vi "Update Methods Registration.vi"(8 "error in (no error)":errorcluster, 11 "Server class in":refnum<vi>) -> (0 "error out":errorcluster, 3 "Server class out":refnum<vi>)   [LabVIEW 2019, in "gRPC Template Creation Utility.lvlib"]
uses:
  gRPC Template Creation Utility.lvlib
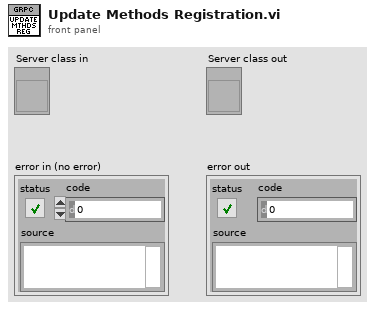
[diagram p1: front panel]
types:
  T1 = typedef "LVPointTypeDef.ctl" = cluster{"Horizontal":i16, "Vertical":i16}
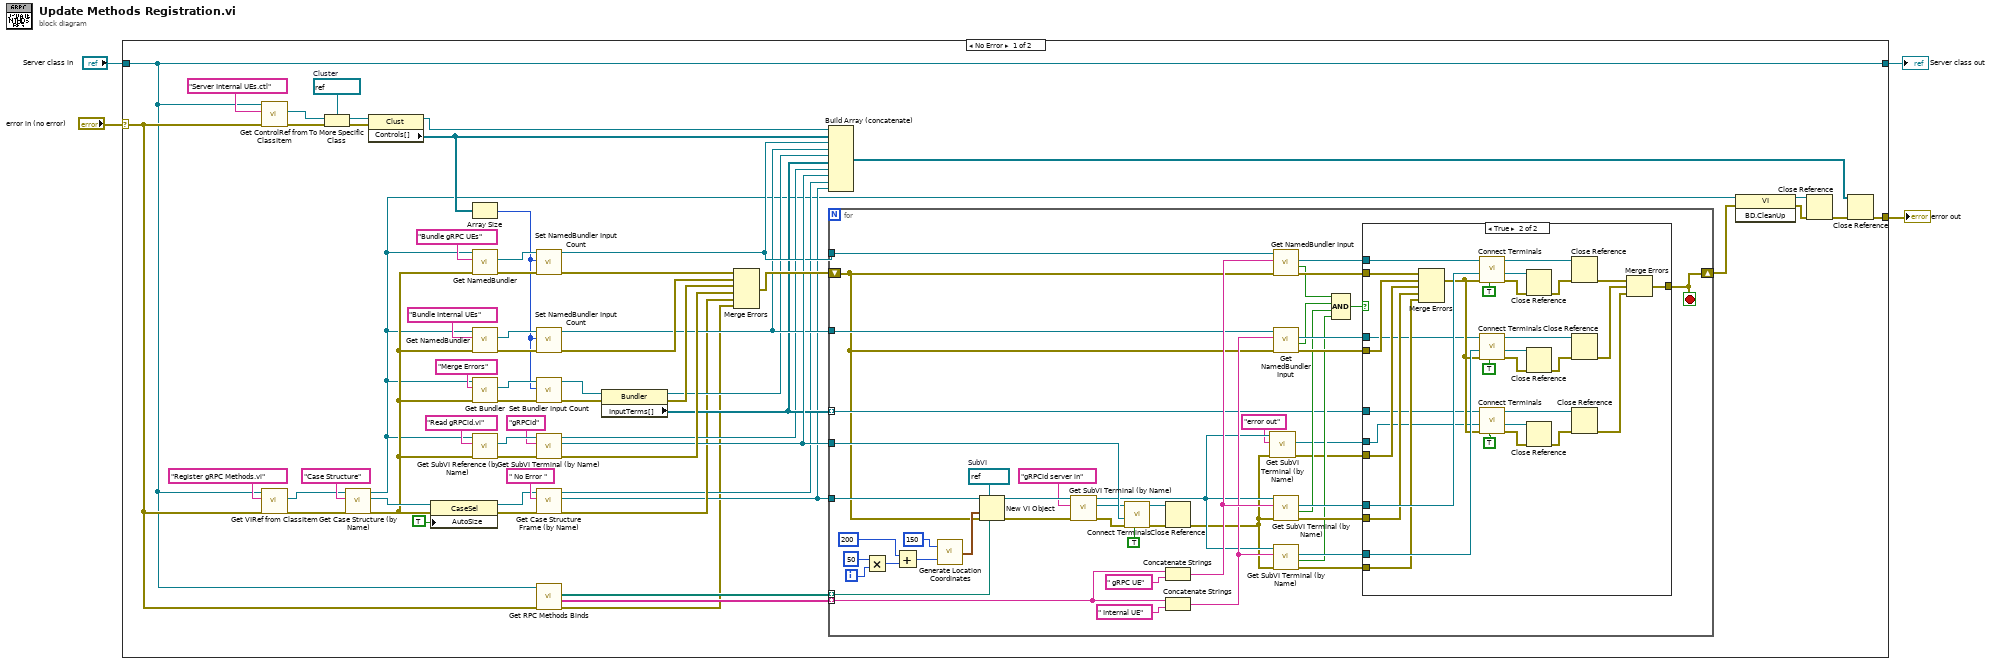
[diagram p0: block diagram]
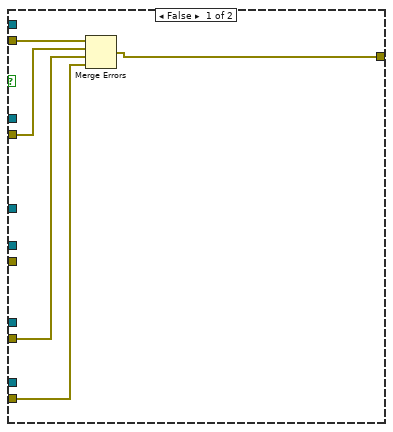
[diagram p2: hidden frame]
diagram:
  n1 = case shown="No Error" "error in (no error)" {
    selector: "error in (no error)" -> [w37 w141]
    tunnel: [w16 w141] -> w4
    tunnel: "Server class in" -> [w36 w142]
    tunnel: [w36 w142] -> w1
    frame No Error {
      w58 = refnum<vi> refnum  # Cluster
      n2 = call "Get ControlRef from ClassItem.vi"("error in (no error)"=w37, "Item Name"="Server Internal UEs.ctl", "LVClassLibrary in"=w36) -> ("error out"=w59:errorcluster, "Control ref out"=w57:refnum<vi>)  [unwired: 5 in, 2 out]
      n3 = call "Get VIRef from ClassItem.vi"("error in (no error)"=w37, "Item Name"="Register gRPC Methods.vi", "LVClassLibrary in"=w36) -> ("error out"=w53:errorcluster, "VIref out"=w33:refnum<vi>)  [unwired: 5 in, 2 out]
      n4 = To More Specific Class(target class=w58, reference=w57, error in=w59) -> (specific class reference=w60:refnum<vi>, error out=w61:errorcluster)
      n5 = call "Get Case Structure (by Name).vi"("error in (no error)"=w53, "Case Structure name"="Case Structure" ("y"), "VI ref in"=w33) -> ("error out"=w28:errorcluster, "CaseStructure out"=w43:refnum<vi>, "VI ref out"=w6:refnum<vi>)  [unwired: 5 in, 1 out]
      n6 = property class="Clust"(reference=w60, error in=w61) -> (reference out=w21:refnum<vi>, "Controls[]"=w20:refnum<vi>[])  [unwired: 1 out]
      n7 = property class="CaseSel"(reference=w43, error in=w28, "AutoSize"=TRUE ("AutoSize To Fit Contents?")) -> (reference out=w42:refnum<vi>, error out=w41:errorcluster)
      n8 = Array Size(array=w20) -> (size(s)=w30:i32)
      n9 = call "Get NamedBundler.vi"("error in (no error)"=w28, "Label"="Bundle gRPC UEs" ("name/order"), "Owner VI in"=w6) -> ("error out"=w51:errorcluster, "NamedBundler ref out"=w63:refnum<vi>)  [unwired: 5 in, 2 out]
      n10 = call "Get NamedBundler.vi"("error in (no error)"=w28, "Label"="Bundle Internal UEs" ("name/order"), "Owner VI in"=w6) -> ("error out"=w49:errorcluster, "NamedBundler ref out"=w50:refnum<vi>)  [unwired: 5 in, 2 out]
      n11 = call "Get Bundler.vi"("error in (no error)"=w28, "label"="Merge Errors" ("Label"), "owner vi in"=w6) -> ("error out"=w27:errorcluster, "bundler ref"=w31:refnum<vi>)  [unwired: 5 in, 2 out]
      n12 = call "Get SubVI Reference (by Name).vi"("error in (no error)"=w28, "SubVI Name"="Read gRPCid.vi", "Owner VI in"=w6) -> ("error out"=w46:errorcluster, "SubVI Refnum out"=w47:refnum<vi>)  [unwired: 5 in, 2 out]
      n13 = call "Set NamedBundler Input Count.vi"("error in (no error)"=w51, "Numeric"=w30, "NamedBundler in"=w63) -> ("error out"=w23:errorcluster, "NamedBundler out"=w14:refnum<vi>)  [unwired: 7 in]
      n14 = call "Set NamedBundler Input Count.vi"("error in (no error)"=w49, "Numeric"=w30, "NamedBundler in"=w50) -> ("error out"=w44:errorcluster, "NamedBundler out"=w13:refnum<vi>)  [unwired: 7 in]
      n15 = call "Set Bundler Input Count.vi"("error in (no error)"=w27, "Numeric"=w30, "Bundler in"=w31) -> ("error out"=w26:errorcluster, "Bundler out"=w29:refnum<vi>)  [unwired: 7 in]
      n16 = call "Get SubVI Terminal (by Name).vi"("error in (no error)"=w46, "Terminal name"="gRPCid", "SubVI in"=w47) -> ("error out"=w24:errorcluster, "SubVI Term ref"=w19:refnum<vi>, "SubVI out"=w10:refnum<vi>)  [unwired: 5 in, 1 out]
      n17 = call "Get Case Structure Frame (by Name).vi"("error in (no error)"=w41, "element"=" No Error ", "CaseStructure in"=w42) -> ("error out"=w9:errorcluster, "Frame ref out"=w8:refnum<vi>, "CaseStructure out"=w7:refnum<vi>)  [unwired: 5 in, 1 out]
      n18 = call "Get RPC Methods Binds.vi"("error in (no error)"=w37, "LVClassLibrary in"=w36) -> ("error out"=w5:errorcluster, "RPC Method Binds Names"=w34:string[], "RPC Method Binds Paths"=w35:path[])  [unwired: 6 in, 1 out]
      n19 = property class="Bundler"(reference=w29, error in=w26) -> (reference out=w12:refnum<vi>, error out=w25:errorcluster, "InputTerms[]"=w11:refnum<vi>[])
      n20 = Merge Errors(w23, w44, w25, w24, w9, w5) -> (w22:errorcluster)
      n21 = Build Array (concatenate)(w21, w20, w14, w13, w12, w11, w10, w19, w7, w8) -> (w15:refnum<vi>[])
      n22 = for {
        tunnel: w8 -> [w110]
        tunnel: w14 -> [w109]
        tunnel: w13 -> [w101]
        tunnel: w19 -> [w85]
        tunnel: w35 -> [w74] mode=indexing
        tunnel: w34 -> [w73] mode=indexing
        tunnel: w11 -> [w68] mode=indexing
        shift-right: [w94] -> w18
        shift-left: w22 -> [w66]
        i -> [w83]
        stop <- w94 stop-if-true
        w108 = refnum<vi> refnum  # SubVI
        n23 = Multiply(x=50 ("y"), y=w83) -> (x*y=w81:i32)
        n24 = Add(x=i16 200 ("Horizontal"), y=w81) -> (x+y=w79:i32)
        n25 = call "Generate Location Coordinates.vi"("Vertical"=w79, "Horizontal"=i16 150) -> ("Location out"=w78:T1)
        n26 = New VI Object(vi object class=w108, owner refnum=w110, position/next to=w78, 6:w74, 8:w66) -> (object refnum=w87:refnum<vi>, 0:w88:errorcluster)  [unwired: 3 in]
        n27 = call "Get SubVI Terminal (by Name).vi"("error in (no error)"=w88, "Terminal name"="gRPCid server in", "SubVI in"=w87) -> ("error out"=w75:errorcluster, "SubVI Term ref"=w76:refnum<vi>, "SubVI out"=w72:refnum<vi>)  [unwired: 5 in, 1 out]
        n28 = call "Connect Terminals.vi"("Auto Route? (F)"=TRUE, "Error In"=w75, "Source Terminal"=w85, "Sink Terminal"=w76) -> ("Error Out"=w65:errorcluster)  [unwired: 7 in]
        n29 = Close Reference(reference=w76, error in (no error)=w65) -> (error out=w70:errorcluster)
        n30 = Concatenate Strings(w73, " gRPC UE" ("string")) -> (w104:string)
        n31 = Concatenate Strings(w73, " Internal UE" ("string")) -> (w102:string)
        n32 = call "Get SubVI Terminal (by Name).vi"("error in (no error)"=w70, "Terminal name"="error out", "SubVI in"=w72) -> ("error out"=w69:errorcluster, "SubVI Term ref"=w67:refnum<vi>)  [unwired: 5 in, 2 out]
        n33 = call "Get NamedBundler Input.vi"("error in (no error)"=w66, "Input name"=w104, "NamedBundler ref in"=w109) -> ("error out"=w98:errorcluster, "Found?"=w93:bool, "Input Term ref"=w107:refnum<vi>)  [unwired: 5 in, 1 out]
        n34 = call "Get NamedBundler Input.vi"("error in (no error)"=w66, "Input name"=w102, "NamedBundler ref in"=w101) -> ("error out"=w96:errorcluster, "Found?"=w92:bool, "Input Term ref"=w100:refnum<vi>)  [unwired: 5 in, 1 out]
        n35 = call "Get SubVI Terminal (by Name).vi"("error in (no error)"=w70, "Terminal name"=w104, "SubVI in"=w72) -> ("error out"=w97:errorcluster, "Found?"=w91:bool, "SubVI Term ref"=w106:refnum<vi>)  [unwired: 5 in, 1 out]
        n36 = call "Get SubVI Terminal (by Name).vi"("error in (no error)"=w70, "Terminal name"=w102, "SubVI in"=w72) -> ("error out"=w95:errorcluster, "Found?"=w90:bool, "SubVI Term ref"=w99:refnum<vi>)  [unwired: 5 in, 1 out]
        n37 = Compound Arithmetic op=AND(w93, w92, w91, w90) -> (w89:bool)
        n38 = case shown="True" w89 {
          tunnel: w107 -> [_ w119]
          tunnel: w106 -> [_ w137]
          tunnel: w100 -> [_ w122]
          tunnel: w99 -> [_ w136]
          tunnel: w98 -> [w115 w135]
          tunnel: w97 -> [w112 w132]
          tunnel: w96 -> [w113 w134]
          tunnel: w95 -> [w111 w131]
          tunnel: [w114 w140] -> w94
          tunnel: w69 -> [_ w133]
          tunnel: w68 -> [_ w127]
          tunnel: w67 -> [_ w125]
          frame False {
            n39 = Merge Errors(w115, w113, w112, w111) -> (w114:errorcluster)
          }
          frame True {
            n40 = Merge Errors(w135, w134, w133, w132, w131) -> (w129:errorcluster)
            n41 = call "Connect Terminals.vi"("Auto Route? (F)"=TRUE, "Error In"=w129, "Source Terminal"=w137, "Sink Terminal"=w119) -> ("Error Out"=w117:errorcluster)  [unwired: 7 in]
            n42 = call "Connect Terminals.vi"("Auto Route? (F)"=TRUE, "Error In"=w129, "Source Terminal"=w136, "Sink Terminal"=w122) -> ("Error Out"=w123:errorcluster)  [unwired: 7 in]
            n43 = call "Connect Terminals.vi"("Auto Route? (F)"=TRUE, "Error In"=w129, "Source Terminal"=w125, "Sink Terminal"=w127) -> ("Error Out"=w126:errorcluster)  [unwired: 7 in]
            n44 = Close Reference(reference=w137, error in (no error)=w117) -> (error out=w118:errorcluster)
            n45 = Close Reference(reference=w136, error in (no error)=w123) -> (error out=w121:errorcluster)
            n46 = Close Reference(reference=w125, error in (no error)=w126) -> (error out=w128:errorcluster)
            n47 = Close Reference(reference=w119, error in (no error)=w118) -> (error out=w116:errorcluster)
            n48 = Close Reference(reference=w122, error in (no error)=w121) -> (error out=w120:errorcluster)
            n49 = Close Reference(reference=w127, error in (no error)=w128) -> (error out=w124:errorcluster)
            n50 = Merge Errors(w116, w120, w124) -> (w140:errorcluster)
          }
        }
      }
      n51 = invoke class="VI" method="BD.CleanUp"(reference=w6, error in=w18) -> (reference out=w39:refnum<vi>, error out=w38:errorcluster)  [unwired: 1 in, 1 out]
      n52 = Close Reference(reference=w39, error in (no error)=w38) -> (error out=w17:errorcluster)
      n53 = Close Reference(reference=w15, error in (no error)=w17) -> (error out=w16:errorcluster)
    }
    frame Error {
    }
  }
  "error out" <- w4
  "Server class out" <- w1
